vi "lab2.vi"() -> ()   [LabVIEW 2026]
panel:
  out "Peak to Peak":dbl
  out "Positive Peak":dbl
  out "data":dynamicdata(graph)
  in  "stop (F)":bool
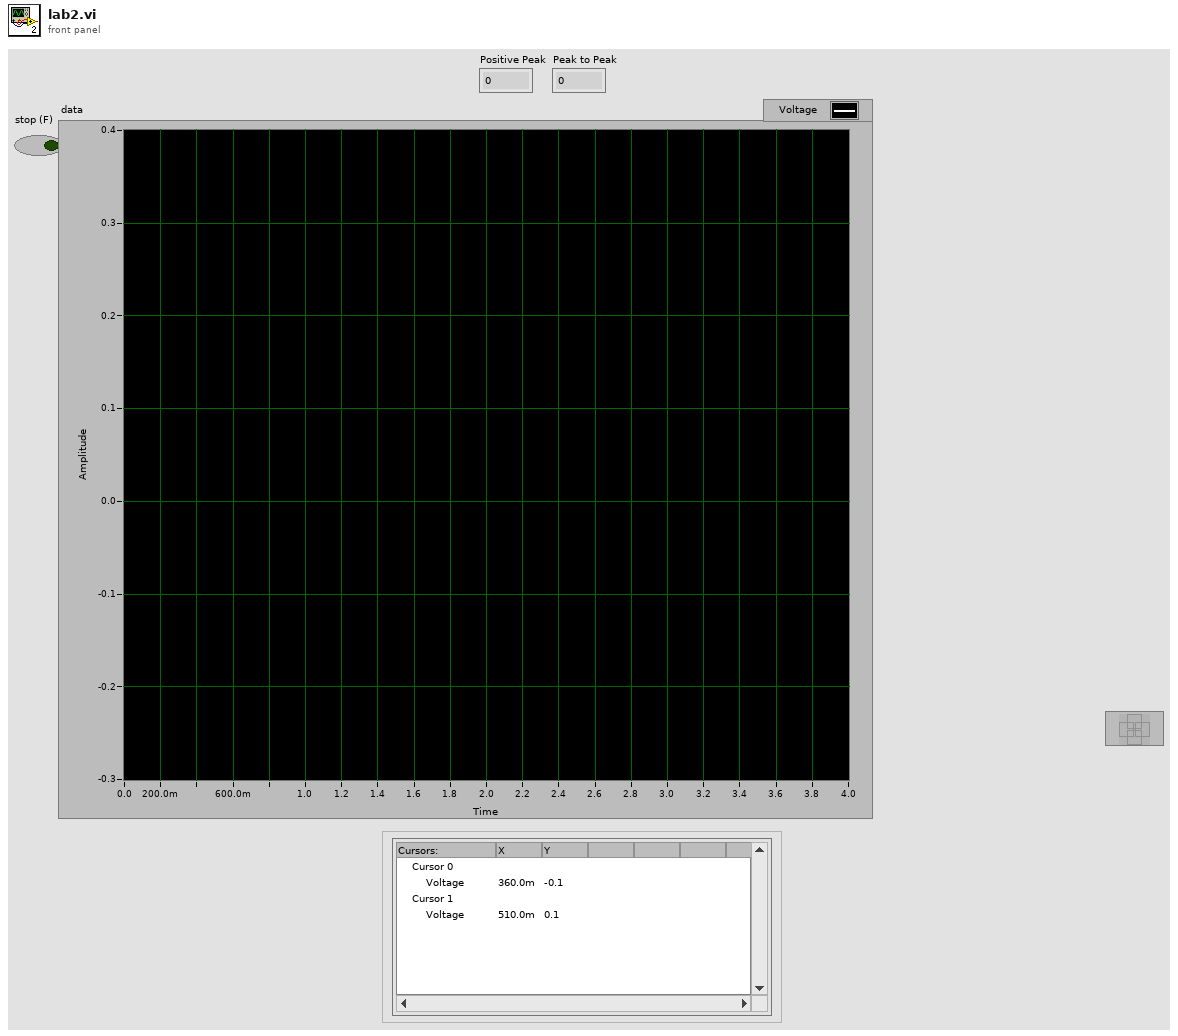
[diagram p1: front panel]
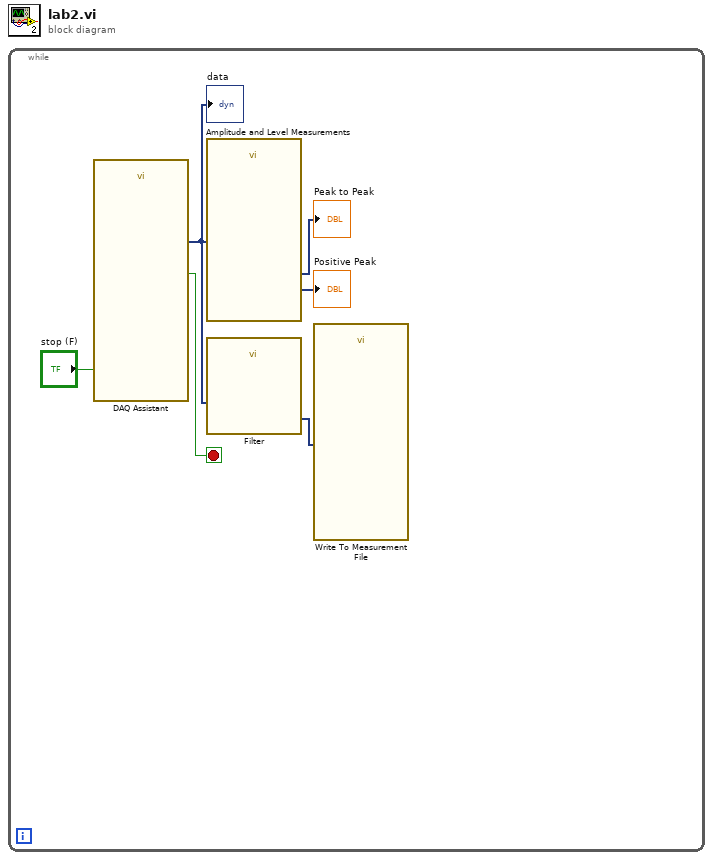
[diagram p0: block diagram]
diagram:
  n1 = while {
    stop <- w5 stop-if-true
    n2 = call "DAQ Assistant"("stop (F)"="stop (F)") -> ("data"=w2:dynamicdata, "stopped"=w5:bool)  [unwired: 15 in, 2 out]
    "data" <- w2
    n3 = call "Amplitude and Level Measurements"("Signals"=w2) -> ("Positive Peak"=→"Positive Peak":dynamicdata, "Peak to Peak"=→"Peak to Peak":dynamicdata)  [unwired: 10 in, 3 out]
    n4 = call "Filter"("Signal"=w2) -> ("Filtered Signal"=w1:dynamicdata)  [unwired: 9 in, 1 out]
    n5 = call "Write To Measurement File"("Signals"=w1) -> ()  [unwired: 16 in, 3 out]
  }
